vi "VIH Utility - UI - Drag and Drop Supporter (w Symbol Indices).vi"(6 "Cmd":enum16{"make symbols", "test D'n'D"}(ring), 11 "Item Symbols":i32[](array[numeric])) -> (0 "an item dragged":bool, 2 "indices":i32[](array[numeric]), 3 "Item Symbols out":i32[](array[numeric]))   [LabVIEW 2014]
doc: "::: VI Helpeks :::\nCopyright (c) 2000-2026 Konstantin Shifershteyn. All rights reserved."
panel:
  # "VI Helpeks\nCopyright (c) 2012-2026 Konstantin Shifershteyn"
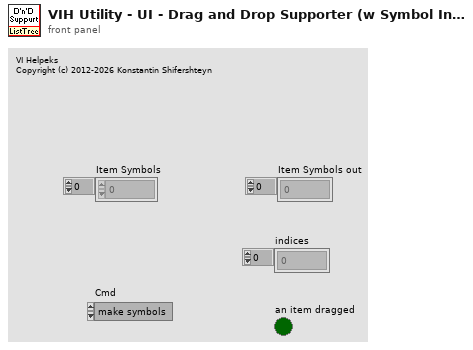
[diagram p1: front panel]
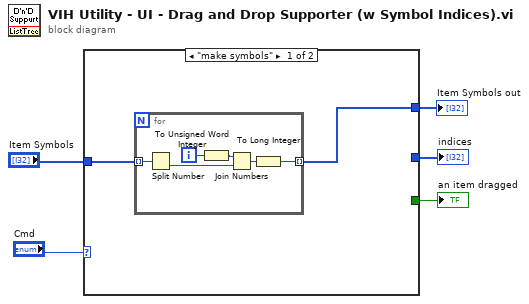
[diagram p0: block diagram]
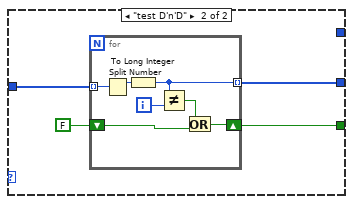
[diagram p2: hidden frame]
diagram:
  n1 = case shown="\"make symbols\"" "Cmd" {
    tunnel: "Item Symbols" -> [w7 w17]
    tunnel: [_ w15] -> w5
    tunnel: [_ w14] -> w4
    tunnel: [w6 _] -> w2
    frame "make symbols" {
      n2 = for {
        tunnel: w7 -> [w13] mode=indexing
        tunnel: [w8] -> w6 mode=indexing
        i -> [w10]
        n3 = Split Number(x=w13) -> (lo(x)=w12:u16)  [unwired: 1 out]
        n4 = To Unsigned Word Integer(number=w10) -> (unsigned 16bit integer=w11:u16)
        n5 = Join Numbers(hi=w11, lo=w12) -> ((hi.lo)=w9:u32)
        n6 = To Long Integer(number=w9) -> (32bit integer=w8:i32)
      }
    }
    frame "test D'n'D" {
      n7 = for {
        tunnel: w17 -> [w24] mode=indexing
        shift-right: [w22] -> w15
        shift-left: FALSE -> [w20]
        tunnel: [w19] -> w14 mode=indexing
        i -> [w18]
        n8 = Split Number(x=w24) -> (hi(x)=w23:u16)  [unwired: 1 out]
        n9 = To Long Integer(number=w23) -> (32bit integer=w19:i32)
        n10 = Not Equal?(x=w19, y=w18) -> (x != y?=w21:bool)
        n11 = Or(x=w21, y=w20) -> (x .or. y?=w22:bool)
      }
    }
  }
  "an item dragged" <- w5
  "indices" <- w4
  "Item Symbols out" <- w2
